vi "Launch Standard Configuration Editor.vi"   [LabVIEW 2013]
uses:
  <vilib>/NI/Progress Bar/Controls/Update Bar Actions.ctl
  <vilib>/NI/Progress Bar/Controls/Progress Bar Properties.ctl
  Standard Editor/Configuration Utility.vi
  <vilib>/NI/Progress Bar/Progress Bar.lvlib
  Standard Editor/Standard Editor.lvlib
types:
  T1 = typedef "Progress Bar.lvlib/Progress Bar Properties.ctl" = cluster{"Background Color":u32, "Installer Title":string, "Title Color":u32, "Action Text":string, "Text Color":u32, "Slider Value":u8, "Bar Color":u32, "Timeout":i32}
  T2 = typedef "Progress Bar.lvlib/Update Bar Actions.ctl" = enum16{"Add To Existing", "Set to Value"}
  T3 = enum32{"Invalid", "Standard", "Closed", "Hidden", "Minimized", "Maximized"}
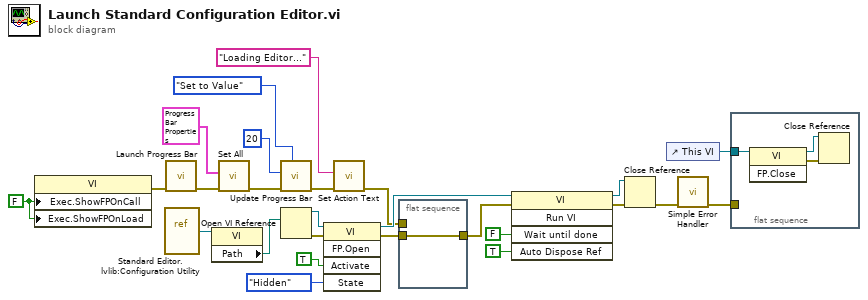
[diagram p0: block diagram]
diagram:
  w2 = FALSE ("Execution:Show Front Panel On Call")
  n1 = property class="VI"("Exec.ShowFPOnCall"=w2, "Exec.ShowFPOnLoad"=w2) -> (error out=w1:errorcluster)  [unwired: 2 in, 1 out]
  n2 = vi-ref "Standard Editor.lvlib:Configuration Utility.vi"() -> (w5:refnum<vi>)
  n3 = call <vilib>:"Launch Progress Bar.vi"("error in (no error)"=w1) -> ("error out"=w12:errorcluster)  [unwired: 9 in, 1 out]
  n4 = property class="VI"(reference=w5) -> ("Path"=w4:path)  [unwired: 1 in, 2 out]
  n5 = call <vilib>:"Set All.vi"("error in (no error)"=w12, "Progress Bar Properties (Default)"=T1 {"Background Color"=3381759, "Installer Title"="LabVIEW DCAF", "Title Color"=0, "Action Text"="", "Text Color"=0, "Slider Value"=0, "Bar Color"=6618880, "Timeout"=0}) -> ("error out"=w11:errorcluster)  [unwired: 9 in]
  n6 = call <vilib>:"Update Progress Bar.vi"("Action"=Update_Bar_Actions."Set to Value", "error in (no error)"=w11, "Value"=u8 20) -> ("error out"=w9:errorcluster)  [unwired: 8 in]
  n7 = Open VI Reference(vi path=w4) -> (vi reference=w25:refnum<vi>, error out=w26:errorcluster)  [unwired: 5 in]
  n8 = invoke class="VI" method="FP.Open"(reference=w25, error in=w26, "Activate"=TRUE ("Activate?"), "State"=T3."Hidden") -> (reference out=w20:refnum<vi>, error out=w13:errorcluster)  [unwired: 1 in, 3 out]
  n9 = call <vilib>:"Set Action Text.vi"("error in (no error)"=w9, "Action Text"="Loading Editor...") -> ("error out"=w7:errorcluster)  [unwired: 9 in]
  n10 = flat-sequence {
    tunnel: [w27] -> w14
    tunnel: w13 -> [w27]
    tunnel: w7 -> [_]
    frame #0 {
    }
  }
  n11 = invoke class="VI" method="Run VI"(reference=w20, error in=w14, "Wait until done"=FALSE ("Wait Until Done"), "Auto Dispose Ref"=TRUE ("Auto Dispose Reference")) -> (reference out=w19:refnum<vi>, error out=w21:errorcluster)  [unwired: 1 in, 3 out]
  n12 = Close Reference(reference=w19, error in (no error)=w21) -> (error out=w22:errorcluster)
  n13 = control-ref of="This VI"() -> (w17:refnum<vi>)
  n14 = call <vilib>:"Simple Error Handler.vi"("error in (no error)"=w22) -> ("error out"=w18:errorcluster)  [unwired: 4 in, 4 out]
  n15 = flat-sequence {
    tunnel: w18 -> [_]
    tunnel: w17 -> [w28]
    frame #0 {
      n16 = invoke class="VI" method="FP.Close"(reference=w28) -> (reference out=w29:refnum<vi>, error out=w30:errorcluster)  [unwired: 2 in, 1 out]
      n17 = Close Reference(reference=w29, error in (no error)=w30) -> ()  [unwired: 1 out]
    }
  }
